vi "Main.vi"() -> ()   [LabVIEW 2018, in "VisitorPatternDemo.lvclass"]
uses:
  VisitorPatternDemo.lvclass
  Dot Class/Dot.lvclass
  C:/Users/fflores/Documents/LabVIEW-Open-Projects/LabIVEW OOP Design Patterns/Visitor Pattern/Shape Class/Shape.lvclass
  Circle Class/Circle.lvclass
  Rectangle Class/Rectangle.lvclass
  CompoundShape Class/CompoundShape.lvclass
  XMLExportVisitor Class/XMLExportVisitor.lvclass
  ConsoleOut/Print Options.ctl
panel:
  out "XML String Exported":string
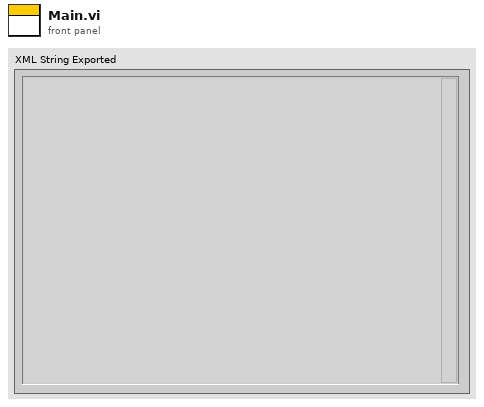
[diagram p1: front panel]
types:
  T1 = typedef "Print Options.ctl" = enum16{"Create", "Get Reference", "Print", "Print Header", "Close"}
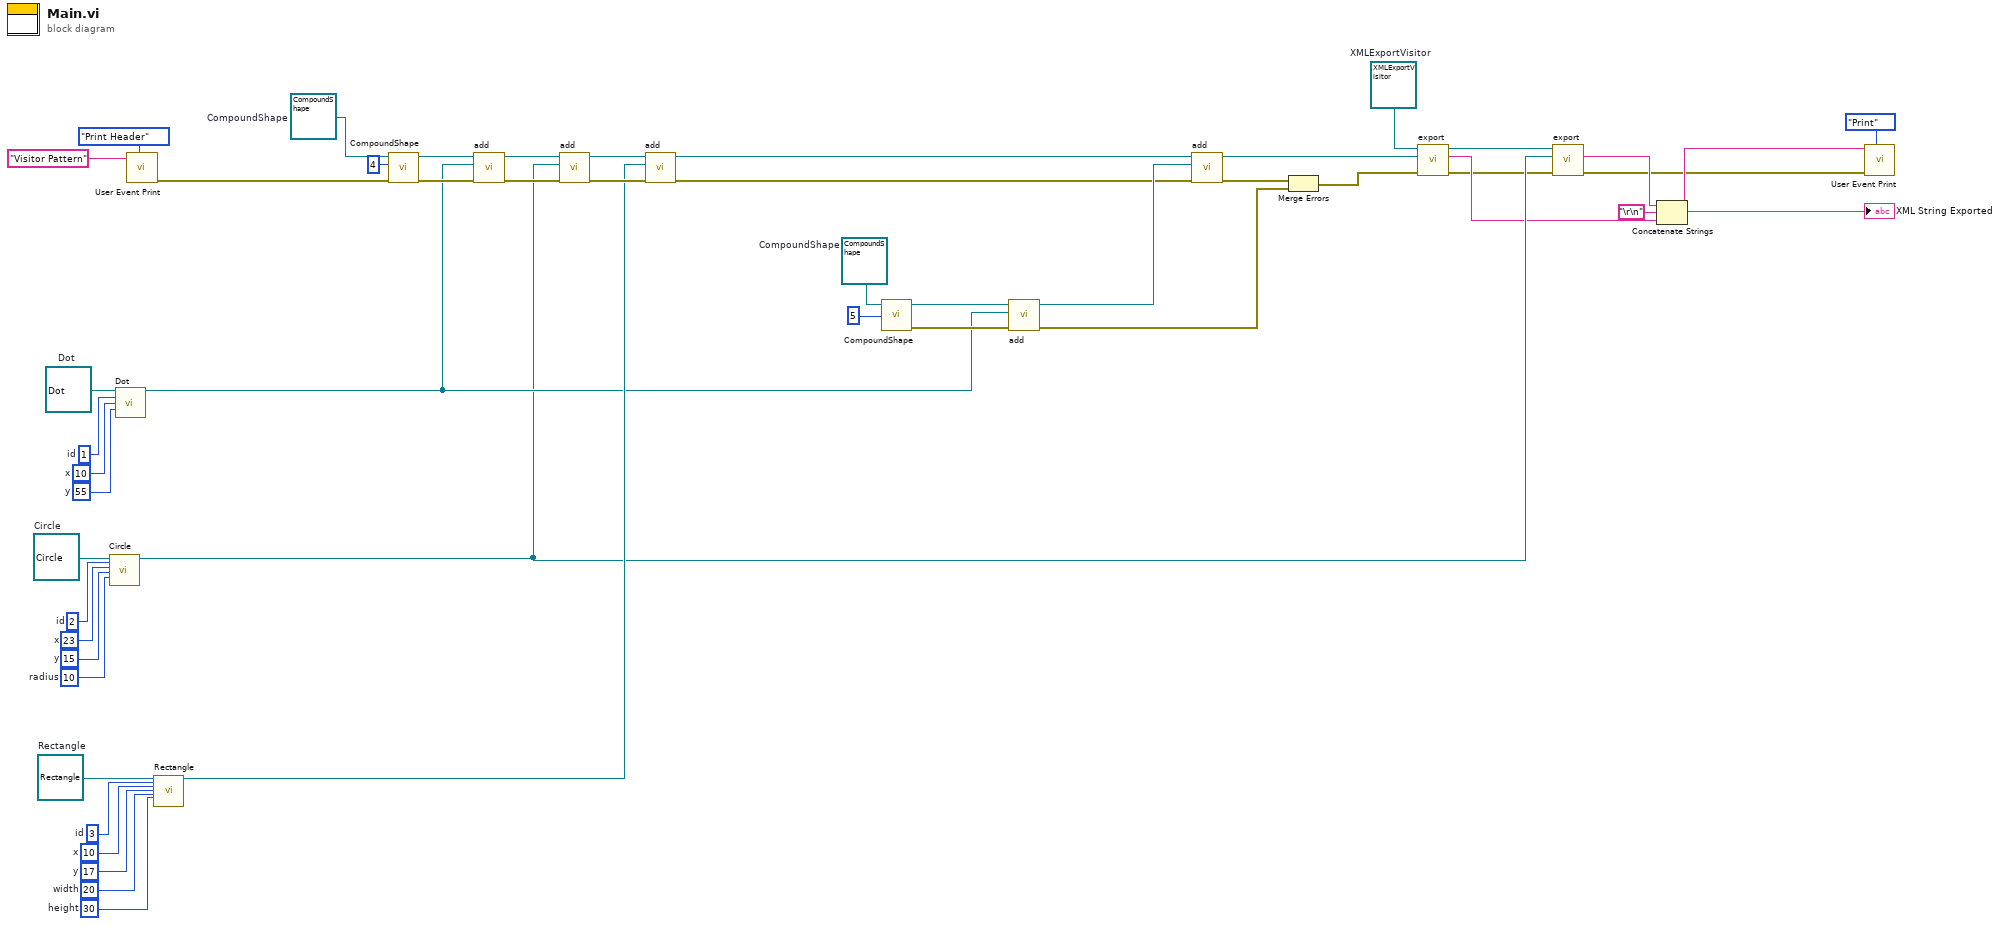
[diagram p0: block diagram]
diagram:
  w20 = refnum<class "XMLExportVisitor.lvclass"> refnum  # XMLExportVisitor
  w24 = refnum<class "CompoundShape.lvclass"> refnum  # CompoundShape
  w35 = 30  # height
  w36 = 20  # width
  w37 = 17  # y
  w38 = 10  # x
  w39 = 3  # id
  w41 = 10  # radius
  w42 = 15  # y
  w43 = 23  # x
  w44 = 2  # id
  w34 = refnum<class "CompoundShape.lvclass"> refnum  # CompoundShape
  w40 = refnum<class "Rectangle.lvclass"> refnum  # Rectangle
  w45 = refnum<class "Circle.lvclass"> refnum  # Circle
  w46 = 55  # y
  w47 = 10  # x
  w48 = 1  # id
  w49 = refnum<class "Dot.lvclass"> refnum  # Dot
  n1 = call "Circle.vi"("Circle in"=w45, "id"=w44, "x"=w43, "y"=w42, "radius"=w41) -> ("Circle out"=w17:refnum<class "Circle.lvclass">)  [unwired: 13 in, 1 out]
  n2 = call "Dot.vi"("Dot in"=w49, "id"=w48, "x"=w47, "y"=w46) -> ("Dot out"=w21:refnum<class "Dot.lvclass">)  [unwired: 10 in, 1 out]
  n3 = call "User Event Print.vi"("Options"=Print_Options."Print Header", "String to Print"="Visitor Pattern") -> ("error out"=w8:errorcluster)  [unwired: 8 in, 1 out]
  n4 = call "Rectangle.vi"("Rectangle in"=w40, "id"=w39, "x"=w38, "y"=w37, "width"=w36, "height"=w35) -> ("Rectangle out"=w26:refnum<class "Rectangle.lvclass">)  [unwired: 20 in, 1 out]
  n5 = call "CompoundShape.vi"("error in (no error)"=w8, "id"=4, "CompoundShape in"=w34) -> ("error out"=w31:errorcluster, "CompoundShape out"=w32:refnum<class "CompoundShape.lvclass">)  [unwired: 7 in]
  n6 = call "add.vi"("error in (no error)"=w31, "Shape"=w21, "CompoundShape in"=w32) -> ("error out"=w29:errorcluster, "CompoundShape out"=w30:refnum<class "CompoundShape.lvclass">)  [unwired: 7 in]
  n7 = call "add.vi"("error in (no error)"=w29, "Shape"=w17, "CompoundShape in"=w30) -> ("error out"=w27:errorcluster, "CompoundShape out"=w28:refnum<class "CompoundShape.lvclass">)  [unwired: 7 in]
  n8 = call "add.vi"("error in (no error)"=w27, "Shape"=w26, "CompoundShape in"=w28) -> ("error out"=w6:errorcluster, "CompoundShape out"=w14:refnum<class "CompoundShape.lvclass">)  [unwired: 7 in]
  n9 = call "CompoundShape.vi"("id"=5, "CompoundShape in"=w24) -> ("error out"=w22:errorcluster, "CompoundShape out"=w23:refnum<class "CompoundShape.lvclass">)  [unwired: 8 in]
  n10 = call "add.vi"("error in (no error)"=w22, "Shape"=w21, "CompoundShape in"=w23) -> ("error out"=w1:errorcluster, "CompoundShape out"=w13:refnum<class "CompoundShape.lvclass">)  [unwired: 7 in]
  n11 = call "add.vi"("error in (no error)"=w6, "Shape"=w13, "CompoundShape in"=w14) -> ("error out"=w2:errorcluster, "CompoundShape out"=w12:refnum<class "CompoundShape.lvclass">)  [unwired: 7 in]
  n12 = Merge Errors(w2, w1) -> (w5:errorcluster)
  n13 = call "export.vi"("error in (no error)"=w5, "Shape"=w12, "XMLExportVisitor in"=w20) -> ("error out"=w4:errorcluster, "String"=w16:string, "XMLExportVisitor out"=w19:refnum<class "XMLExportVisitor.lvclass">)  [unwired: 6 in]
  n14 = call "export.vi"("error in (no error)"=w4, "Shape"=w17, "XMLExportVisitor in"=w19) -> ("error out"=w3:errorcluster, "String"=w18:string)  [unwired: 6 in, 1 out]
  n15 = Concatenate Strings(w18, "\r\n", w16) -> (w11:string)
  "XML String Exported" <- w11
  n16 = call "User Event Print.vi"("Options"=Print_Options."Print", "error in (no error)"=w3, "String to Print"=w11) -> ()  [unwired: 7 in, 2 out]
